vi "Fixture Tab Panel.vi"() -> ()   [LabVIEW 2020]
doc: "Shows how to programmatically manipulate the appearance of a tab control. Specific examples include changing the names of the pages, changing the page enabled state, hiding pages, and coloring individual pages different colors."
panel:
  in  "Tab":enum32{"One", "Two"}(tab)
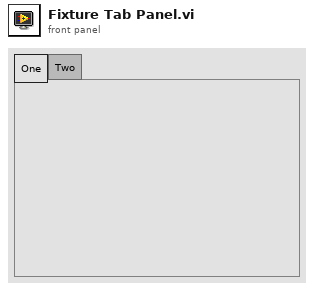
[diagram p1: front panel]
types:
  T1 = enum32{"Page Enabled", "Page Disabled", "Page Disabled & Grayed"}
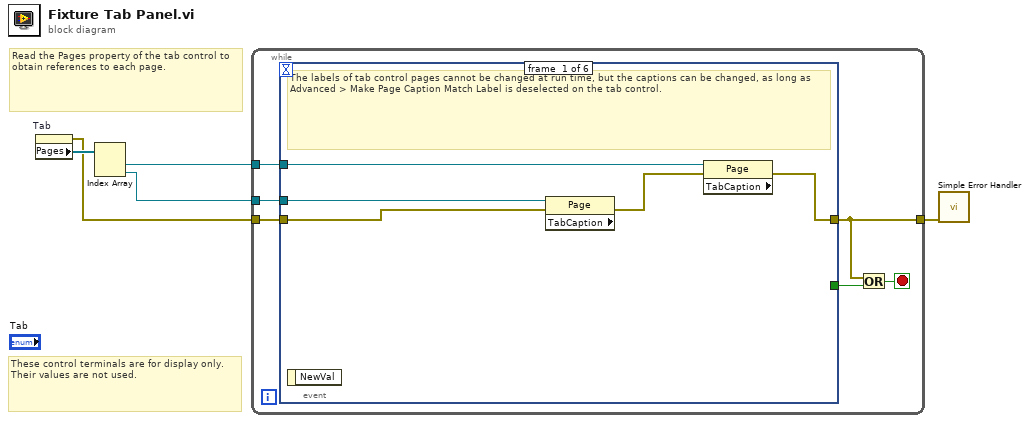
[diagram p0: block diagram]
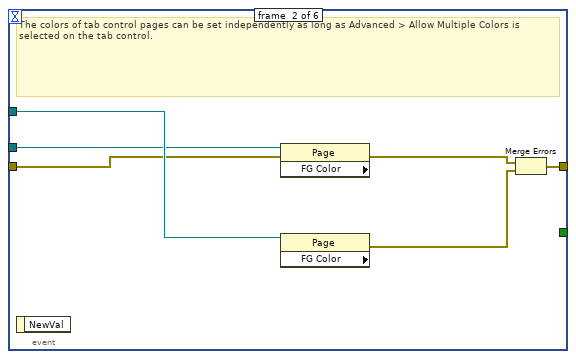
[diagram p2: hidden frame]
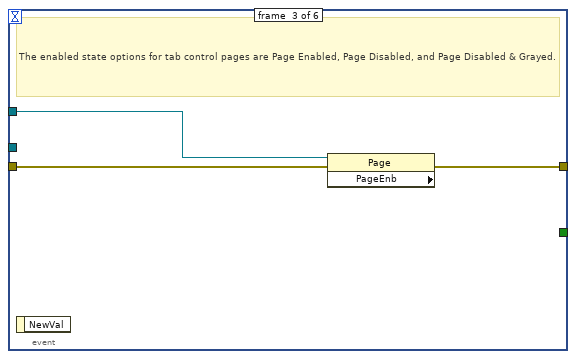
[diagram p3: hidden frame]
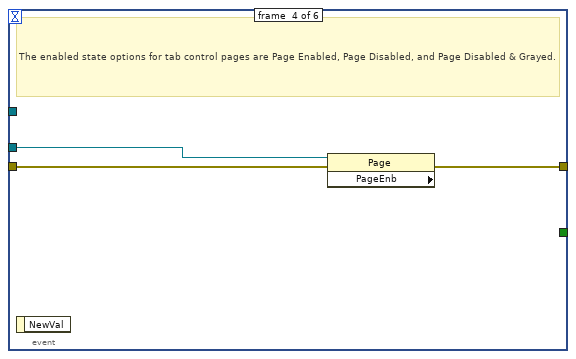
[diagram p4: hidden frame]
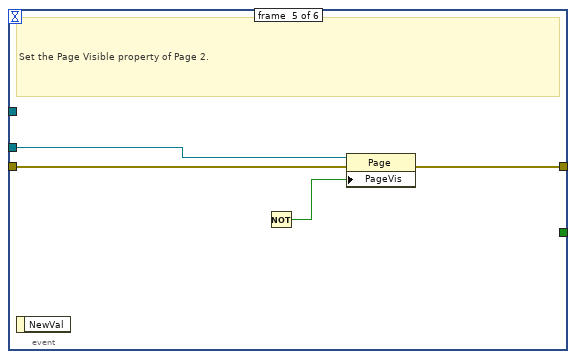
[diagram p5: hidden frame]
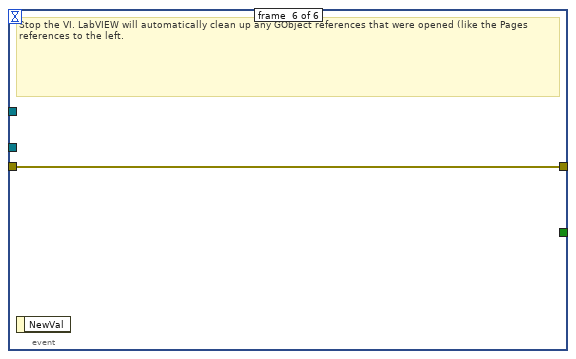
[diagram p6: hidden frame]
diagram:
  # "These control terminals are for display only. Their values are not used."
  # "Read the Pages property of the tab control to obtain references to each page."
  n1 = property on="Tab" class="TabCtl (strict)"() -> (error out=w2:errorcluster, "Pages"=w5:refnum<vi>[])  [unwired: 2 in, 1 out]
  n2 = Index Array(array=w5) -> (element #1=w4:refnum<vi>, element #2=w3:refnum<vi>)  [unwired: 2 in]
  n3 = while {
    tunnel: w4 -> [w10]
    tunnel: w3 -> [w9]
    tunnel: w2 -> [w8]
    tunnel: [w6] -> w1
    stop <- w7 stop-if-true
    n4 = event {
      selector: _ -> [_ _ _ _ _ _]
      dyn-events: _ -> [_ _ _ _ _ _]
      timeout: _ -> [_ _ _ _ _ _]
      tunnel: [_ _ _ _ _ w41] -> w11
      tunnel: w10 -> [w18 w26 w27 _ _ _]
      tunnel: w9 -> [w17 w25 _ w34 w39 _]
      tunnel: w8 -> [w16 w24 w30 w33 w38 w40]
      tunnel: [w14 w19 w29 w32 w37 w40] -> w6
      event #0 {
        # "The labels of tab control pages cannot be changed at run time, but the captions can be changed, as long as Advanced > Make Page Caption Match Label is deselected on the tab control."
        n5 = event-data() -> ()  [unwired: 1 in, 1 out]
        n6 = property class="Page"(reference=w17, error in=w16) -> (error out=w15:errorcluster, "TabCaption"=w12:string)  [unwired: 1 out]
        n7 = property class="Page"(reference=w18, error in=w15) -> (error out=w14:errorcluster, "TabCaption"=w13:string)  [unwired: 1 out]
      }
      event #1 {
        # "The colors of tab control pages can be set independently as long as Advanced > Allow Multiple Colors is selected on the tab control."
        n8 = event-data() -> ()  [unwired: 1 in, 1 out]
        n9 = property class="Page"(reference=w25, error in=w24) -> (error out=w21:errorcluster, "FG Color"=w22:u32)  [unwired: 1 out]
        n10 = property class="Page"(reference=w26) -> (error out=w20:errorcluster, "FG Color"=w23:u32)  [unwired: 1 in, 1 out]
        n11 = Merge Errors(w21, w20) -> (w19:errorcluster)
      }
      event #2 {
        # "The enabled state options for tab control pages are Page Enabled, Page Disabled, and Page Disabled & Grayed."
        n12 = event-data() -> ()  [unwired: 1 in, 1 out]
        n13 = property class="Page"(reference=w27, error in=w30) -> (error out=w29:errorcluster, "PageEnb"=w28:T1)  [unwired: 1 out]
      }
      event #3 {
        # "The enabled state options for tab control pages are Page Enabled, Page Disabled, and Page Disabled & Grayed."
        n14 = event-data() -> ()  [unwired: 1 in, 1 out]
        n15 = property class="Page"(reference=w34, error in=w33) -> (error out=w32:errorcluster, "PageEnb"=w31:T1)  [unwired: 1 out]
      }
      event #4 {
        # "Set the Page Visible property of Page 2."
        n16 = event-data() -> ()  [unwired: 1 in, 1 out]
        n17 = Not() -> (x=w36:bool, .not. x?=w35:bool)
        n18 = property class="Page"(reference=w39, error in=w38, "PageVis"=w35) -> (error out=w37:errorcluster)  [unwired: 1 out]
      }
      event #5 {
        # "Stop the VI. LabVIEW will automatically clean up any GObject references that were opened (like the Pages references to the left."
        n19 = event-data() -> ()  [unwired: 1 in, 1 out]
      }
    }
    n20 = Or(x=w6, y=w11) -> (x .or. y?=w7:bool)
  }
  n21 = call <vilib>:"Simple Error Handler.vi"("error in (no error)"=w1) -> ()  [unwired: 4 in, 5 out]
